vi "test Import Invalid Configuration Files.vi"(8 "error in":errorcluster, 11 "TestCase in":refnum<class "Import.lvclass">) -> (0 "error out":errorcluster, 3 "TestCase out":refnum<class "Import.lvclass">)   [LabVIEW 2020, in "Import.lvclass"]
uses:
  Import.lvclass
  Import.lvclass/Import.ctl
  C:/Program Files/National Instruments/LabVIEW 2026/vi.lib/addons/_JKI Toolkits/VI Tester/TestCase.llb/TestCase.lvclass
  <vilib>/addons/_JKI Toolkits/VI Tester/TestCase.llb/TestCase.lvclass
  Import/ARINC 429 Import.lvlib
  <userlib>/_OpenG.lib/appcontrol/appcontrol.llb/openg_application_control.lvlib
  <vilib>/NI/VeriStand Custom Device Testing Tools/VeriStandTestUtilities/VeriStandTestUtilities.lvlib
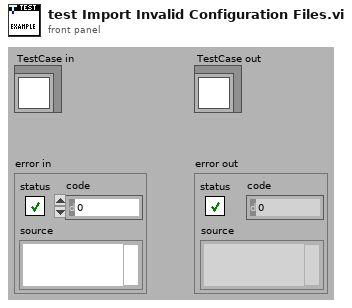
[diagram p1: front panel]
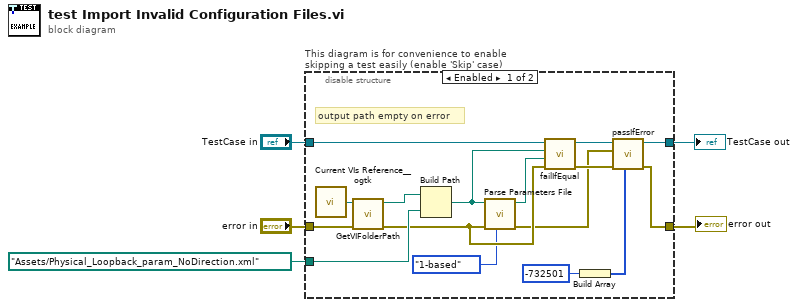
[diagram p0: block diagram]
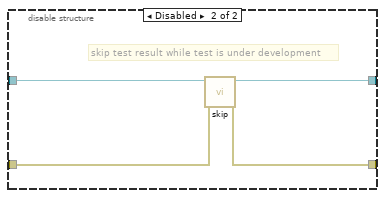
[diagram p2: hidden frame]
diagram:
  n1 = disable-structure "This diagram is for convenience to enable skipping a test easily (enable 'Skip' case)" shown="Enabled" {
    disable-tunnel: "TestCase in" -> [w21 w25]
    disable-tunnel: [w12 w23] -> w2
    disable-tunnel: [w11 w24] -> w4
    disable-tunnel: "error in" -> [w18 w22]
    disable-tunnel: path "Assets/Physical_Loopback_param_NoDirection.xml" ("Absolute or Relative Path") -> [w17 _]
    frame Enabled {
      # "output path empty on error"
      n2 = call <userlib>:"Current VIs Reference__ogtk.vi"() -> ("Current VI's reference"=w20:refnum<vi>)  [unwired: 5 in]
      n3 = call <vilib>:"GetVIFolderPath.vi"("error in (no error)"=w18, "VI Reference in"=w20) -> ("error out"=w13:errorcluster, "VI Folder Path out"=w19:path)  [unwired: 8 in]
      n4 = Build Path(base path=w19, name or relative path=w17) -> (appended path=w16:path)
      n5 = call "Parse Parameters File.vi"("ch indexing (0-based)"=enum16{"0-based", "1-based"}."1-based", "error in"=w13, "path to XML document"=w16) -> ("error out"=w10:errorcluster, "path to XML document out"=w7:path)  [unwired: 6 in, 1 out]
      n6 = call-dynamic "failIfEqual.vi"("error in (no error)"=w13, "y"=w7, "x"=w16, "TestCase in"=w21) -> ("error out"=w14:errorcluster, "TestCase out"=w15:refnum<class "Import.lvclass">)  [unwired: 6 in]
      n7 = Build Array(-732501 ("code")) -> (w8:i32[])
      n8 = call-dynamic "passIfError.vi"("passing error codes (default = any error code)"=w8, "error in (no error)"=w14, "error"=w10, "TestCase in"=w15) -> ("error out"=w11:errorcluster, "TestCase out"=w12:refnum<class "Import.lvclass">)  [unwired: 6 in]
    }
    frame Disabled {
      # "skip test result while test is under development"
      n9 = call <vilib>:"skip.vi"("error in (no error)"=w22, "TestCase in"=w25) -> ("error out"=w24:errorcluster, "TestCase out"=w23:refnum<class "Import.lvclass">)  [unwired: 8 in]
    }
  }
  "error out" <- w4
  "TestCase out" <- w2
